vi "Config_Compile_Plan.vi"(8 "error in (no error)":errorcluster={"status"=FALSE, "code"=0, "source"="\"\""}, 11 "Validated test/group/action tree":string) -> (0 "error out":errorcluster={"status"=FALSE, "code"=0, "source"="\"\""}, 2 "status ok":bool, 3 "Immutable ExecutionPlan":string)   [LabVIEW 2026]
doc: "INTENT: Preprocess definitions for executor. LOGIC: Resolve references and plugins, precompute resource requirements, stable action indexes and branch joins."
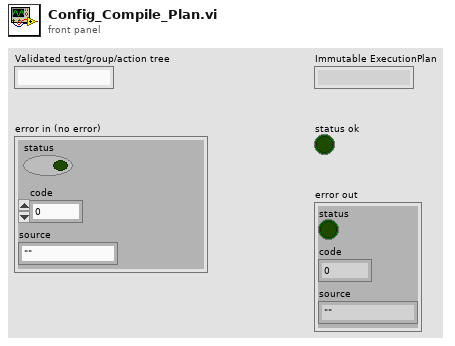
[diagram p1: front panel]
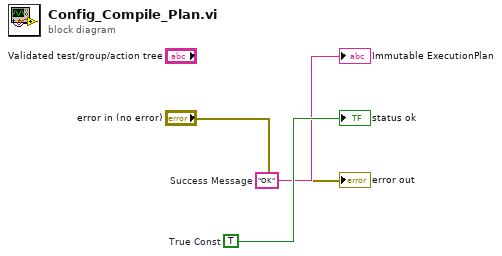
[diagram p0: block diagram]
diagram:
  w3 = TRUE  # True Const
  w2 = "OK"  # Success Message
  "Immutable ExecutionPlan" <- w2
  "status ok" <- w3
  "error out" <- "error in (no error)"
